vi "Check Error and Get Call Result.vi"(7 "AWS Core":refnum<class "HTTP Request.lvclass">, 8 "error in (no error)":errorcluster, 10 "Response body":string, 11 "Response header":string) -> (0 "error out":errorcluster, 1 "Redirect endpoint":string, 2 "500 Or Throttled?":bool=TRUE, 3 "Call Result":string)   [LabVIEW 2015, in "NI_AWS_Core.lvlib" / "HTTP Request.lvclass"]
doc: "Check the respnse header and body if necessary to obtain the call's result (Success or Error codes)."
uses:
  HTTP Request.lvclass
  XML Parsing/NI_XML Parsing.lvlib
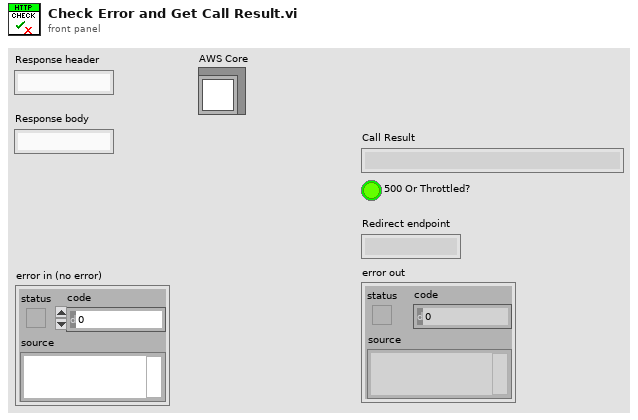
[diagram p1: front panel]
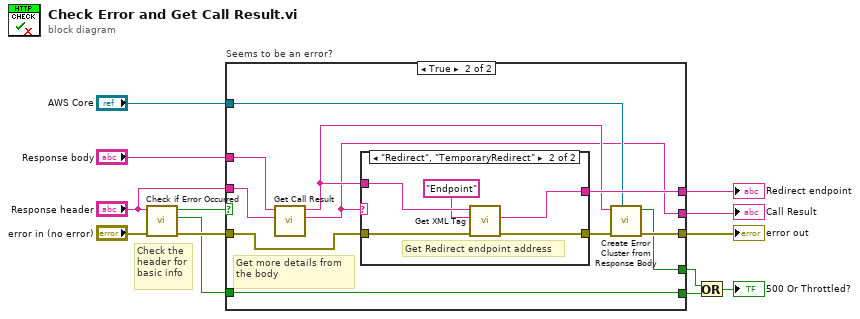
[diagram p0: block diagram]
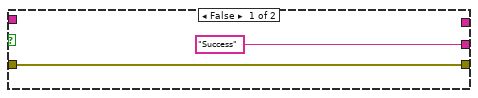
[diagram p2: hidden frame]
diagram:
  # "Check the\nheader for\nbasic info"
  n1 = call "Check if Error Occurred.vi"("error in (no error)"="error in (no error)", "Response header"="Response header") -> ("error out"=w11:errorcluster, "500 Error"=w6:bool, "Error Occurred"=w12:bool)  [unwired: 7 in]
  n2 = case "Seems to be an error?" shown="True" w12 {
    tunnel: w11 -> [w15 w19]
    tunnel: "Response body" -> [_ w18]
    tunnel: [w15 w24] -> w8
    tunnel: ["Success" ("Call Result") w16] -> w9
    tunnel: [_ w26] -> w7
    tunnel: [_ w23] -> w3
    tunnel: [_ w22] -> w5
    tunnel: w6 -> [_ w22]
    tunnel: "AWS Core" -> [_ w21]
    tunnel: "Response header" -> [_ w20]
    frame False {
    }
    frame True {
      # "Get more details from\nthe body"
      n3 = call "Get Call Result.vi"("Response header"=w20, "Response body in"=w18) -> ("Call Result"=w16:string, "Response body out"=w17:string)  [unwired: 8 in]
      n4 = case shown="\"Redirect\", \"TemporaryRedirect\"" w16 {
        tunnel: w17 -> [_ w32]
        tunnel: [_ w30] -> w26
        tunnel: [w27 w29] -> w25
        tunnel: w19 -> [w27 w28]
        frame Default {
        }
        frame "Redirect", "TemporaryRedirect" {
          # "Get Redirect endpoint address"
          n5 = call "Get XML Tag.vi"("error in (no error)"=w28, "Tag name"="Endpoint", "XML String in"=w32) -> ("error out"=w29:errorcluster, "Tag value"=w30:string)  [unwired: 4 in, 3 out]
        }
      }
      n6 = call "Create Error Cluster from Response Body.vi"("AWS Core"=w21, "error in (no error)"=w25, "Response body"=w17) -> ("error out"=w24:errorcluster, "Is Throttled?"=w23:bool)  [unwired: 7 in]
    }
  }
  "Call Result" <- w9
  "error out" <- w8
  "Redirect endpoint" <- w7
  n7 = Or(x=w3, y=w5) -> (x .or. y?=→"500 Or Throttled?":bool)
